vi "clusters.vi"() -> ()   [LabVIEW 2018]
panel:
  in  "Boolean":bool
  in  "Slide":dbl(slide) scale=0.0..100.0
  in  "Slide 2":dbl(slide) scale=0.0..100.0
  out "Cluster 4":T1 {"Gauge" scale=0.0..100.0; "Meter" scale=0.0..100.0}
  out "Cluster 2":T2
  in  "Cluster":T2
  # "Cluster is grouyp data of multiple data type"
  # "controls can be grouped \nindicatos also same\nbut not indicator and control together"
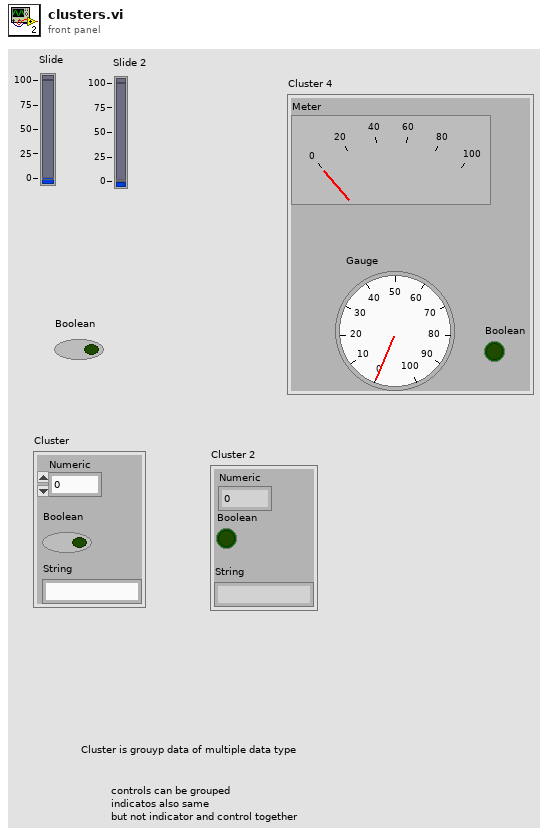
[diagram p1: front panel]
types:
  T1 = cluster{"Meter":dbl, "Gauge":dbl, "Boolean":bool}
  T2 = cluster{"Numeric":dbl, "Boolean":bool, "String":string}
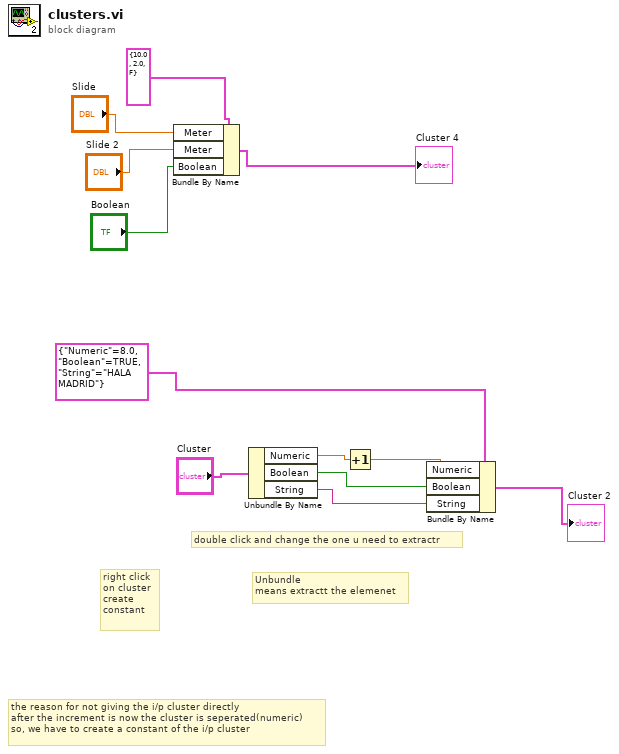
[diagram p0: block diagram]
diagram:
  # "the reason for not giving the i/p cluster directly \nafter the increment is now the cluster is seperated(numeric)\nso, we have to create a constant of the i/p cluster"
  # "right click \non cluster \ncreate \nconstant"
  # "double click and change the one u need to extractr"
  # "Unbundle \nmeans extractt the elemenet"
  n1 = Bundle By Name(cluster=T1 {"Meter"=10.0, "Gauge"=2.0, "Boolean"=FALSE} ("Cluster 4"), "Meter"="Slide", "Meter"="Slide 2", "Boolean"="Boolean") -> (→"Cluster 4":T1)
  n2 = Unbundle By Name("Cluster") -> ("Numeric"=w11:dbl, "Boolean"=w7:bool, "String"=w6:string)
  n3 = Increment(x=w11) -> (x+1=w10:dbl)
  n4 = Bundle By Name(cluster=T2 {"Numeric"=8.0, "Boolean"=TRUE, "String"="HALA MADRID"} ("Cluster"), "Numeric"=w10, "Boolean"=w7, "String"=w6) -> (→"Cluster 2":T2)
